vi "str2str16 - PS.vi"(11 "字符串":string) -> (3 "string":string)   [LabVIEW 2026, in "UI-压力.lvlib" / "Acquisition.lvlib"]
uses:
  Acquisition.lvlib
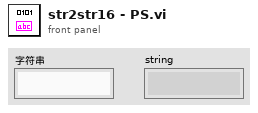
[diagram p1: front panel]
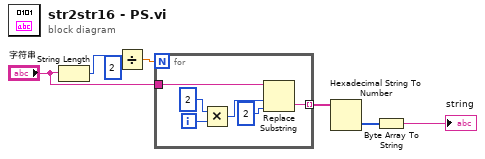
[diagram p0: block diagram]
diagram:
  n1 = String Length(string="字符串") -> (length=w1:i32)
  n2 = Divide(x=w1, y=2) -> (x/y=w3:dbl)
  n3 = for {
    N: w3 -> [_]
    tunnel: "字符串" -> [w9]
    tunnel: [w8] -> w4 mode=indexing
    i -> [w13]
    n4 = Multiply(x=2, y=w13) -> (x*y=w11:i32)
    n5 = Replace Substring(2:2 ("长度（子字符串长度）"), 3:w11, 5:w9) -> (0:w8:string)  [unwired: 1 in, 1 out]
  }
  n6 = Hexadecimal String To Number(string=w4) -> (number=w5:u32[])  [unwired: 2 in, 1 out]
  n7 = Byte Array To String(unsigned byte array=w5) -> (string=→"string":string)
